vi "Quick Stacks - Image Multi Stacks.vi"(7 "Calling VI Ref":refnum<vi>) -> ()   [LabVIEW 2016]
uses:
  <vilib>/Utility/miscctls.llb/LVPointTypeDef.ctl
  Quick Stacks Type Defs/Quick Stack Marked Areas Actions.ctl
  Quick Stacks Type Defs/Quick Stacks Notifier Type.ctl
  Quick Stacks Type Defs/Quick Stack Actions.ctl
  Hardware Configuration/Hardware Configuration Controls/Device Function.ctl
  Hardware Configuration/Hardware Configuration Controls/Device Type.ctl
  Device Library/Stages/Stages Controls/Stage Actions.ctl
  Quick Stacks Type Defs/Quick Stacks Multi Stack Meta Data.ctl
panel:
  out "Current Delay Time (s)":dbl=1.0 format="%.1f"
  out "Current Cycle":u16=1 min=1
  out "XY Positions":cluster{dbl[], dbl[]}[](graph)
  in  "Cycle Delay (s)":u32
  in  "Number of Cycles":u16=1 min=1
  in  "Capture":bool
  in  "Clear All":bool
  in  "Clear Selected":bool
  in  "Mark Point":bool
  in  "Marked Positions":i32(listbox)
  in  "Quit":bool
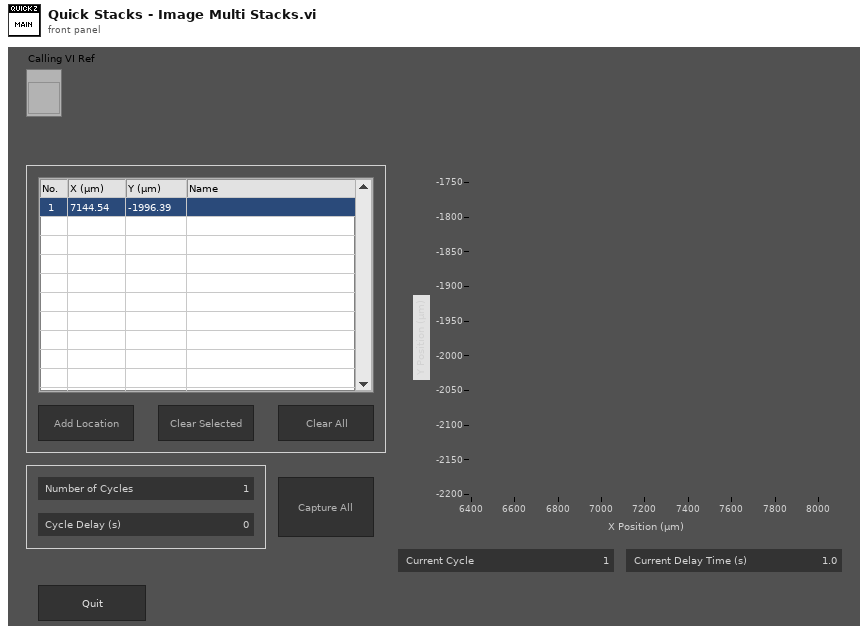
[diagram p1: front panel]
types:
  T1 = typedef "Quick Stacks Notifier Type.ctl" = cluster{"Actions":T2, "Start Z (µm)":dbl, "End Z (µm)":dbl, "Z Size (µm)":dbl, "Num of Steps":u16, "Frames per Step":u16, "Cycle Delay (s)":u32, "Num of Cycles":u16, "Save Path":path, "Running?":bool, "Save File Refs":refnum<file>[]}
  T2 = typedef "Quick Stack Actions.ctl" = enum16{"Idle", "Update Range", "Start Acquisition", "Open File", "Close File", "Start Camera", "Stop Camera", "Laser On", "Laser Off", "Get Image", "Step Z", "Move to Z Start", "Check Cycle", "Abort", "Exit Loop", "Quit"}
  T3 = typedef "Quick Stack Marked Areas Actions.ctl" = enum16{"Add Position", "Update File Name", "Remove Position", "Start Capture", "Move to Position", "Write Meta Data", "Capture", "Switch", "Delay", "Reset Path", "Clear All", "Abort", "Exit Loop", "Quit"}
  T4 = enum16{"Always On", "Always Off", "Off While Running"}
  T5 = typedef "LVPointTypeDef.ctl" = cluster{"Horizontal":i16, "Vertical":i16}
  T6 = typedef "Device Function.ctl" = enum16{"Primary", "Secondary", "Overview", "Wide Field Drift Correction", "642 nm Excitation", "560 nm Excitation", "940 nm Excitation", "546 nm Excitation", "488 nm Excitation", "405 nm Excitation", "Objective Drift Correction", "4Pi Objective Lock", "Objective XY", "Objective Z", "Sample XY", "Sample Coarse Z", "Sample Z", "4Pi Lower", "4Pi Upper", "Mojo", "Adj Cavity", "Line Scanning", "Alert"}
  T7 = typedef "Device Type.ctl" = enum16{"AOTF", "Camera", "Deformable Mirror", "Laser", "Shutter", "Stage", "Waveform", "FPGA", "Email", "Filter Wheel"}
  T8 = typedef "Stage Actions.ctl" = enum16{"Get Position", "MVR", "MOVE", "HALT", "ONTARGET", "ERROR", "REFERENCE", "INIT", "VELOCITY", "STATUS", "EXIT", "HOME", "ZEROPOS", "NANOPOS", "ANALOG", "QUIT"}
  T9 = typedef "Quick Stacks Multi Stack Meta Data.ctl" = cluster{"Start Z (µm)":dbl, "End Z (µm)":dbl, "Z Size (µm)":dbl, "Num of Steps":u16, "Frames per Step":u16, "Cycle Delay (s)":u32, "Num of Cycles":u16}
  T10 = enum32{"Invalid", "Standard", "Closed", "Hidden", "Minimized", "Maximized"}
  T11 = enum8{"Enabled", "Disabled", "Disabled and Grayed Out"}
  T12 = typedef "LVRectTypeDef.ctl" = cluster{"Left":i16, "Top":i16, "Right":i16, "Bottom":i16}
  T13 = typedef "LVBoundsTypeDef.ctl" = cluster{"Width":u32, "Height":u32}
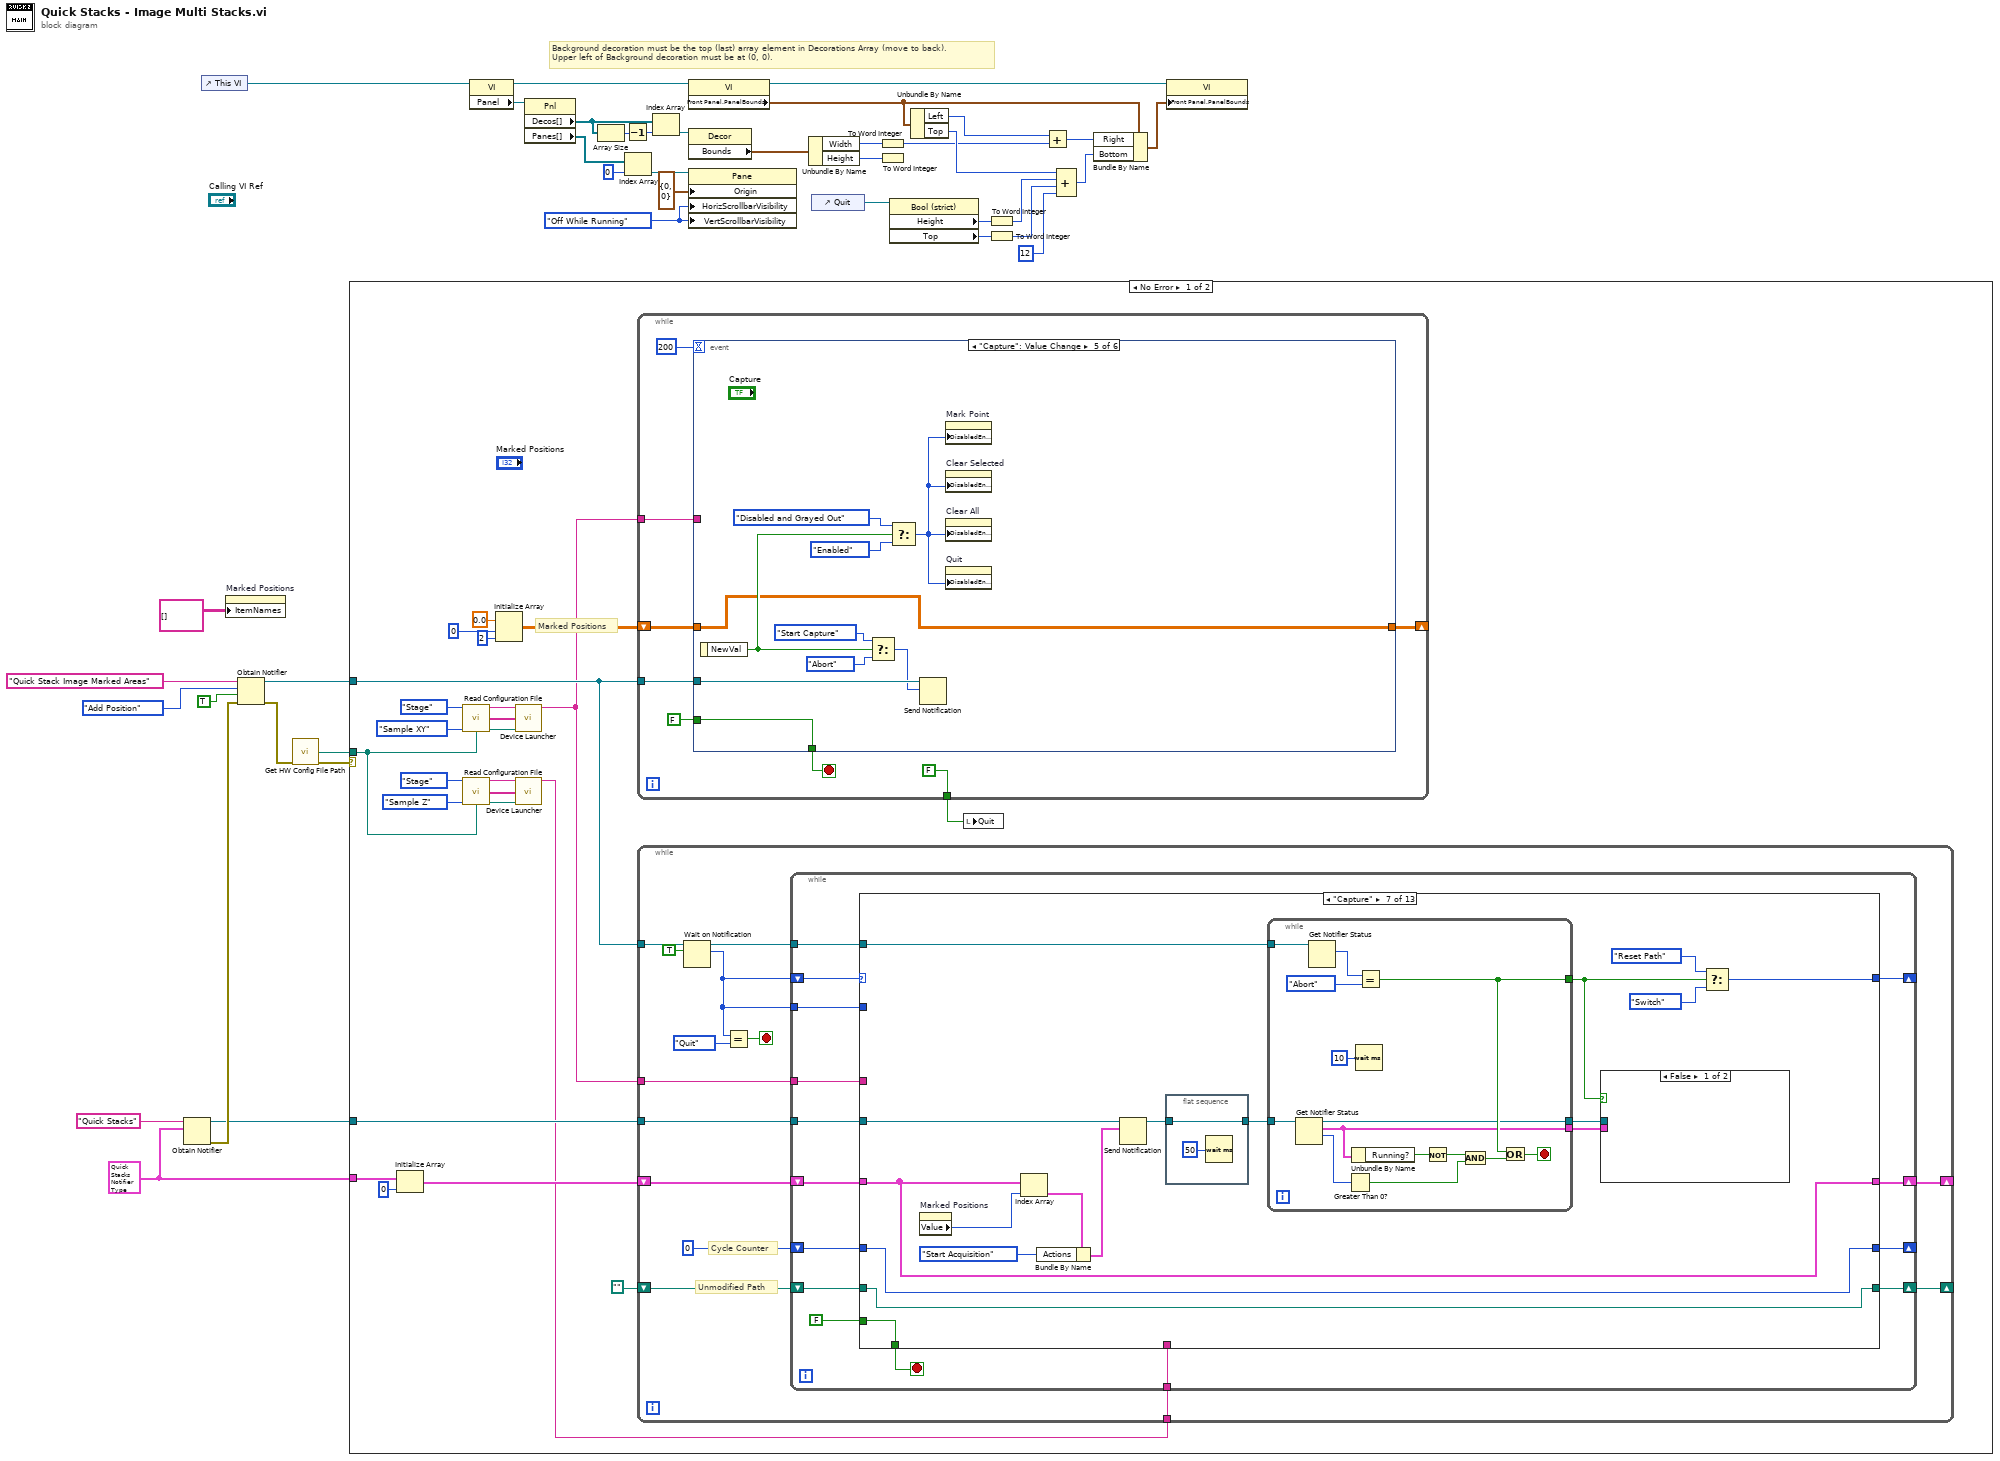
[diagram p0: block diagram]
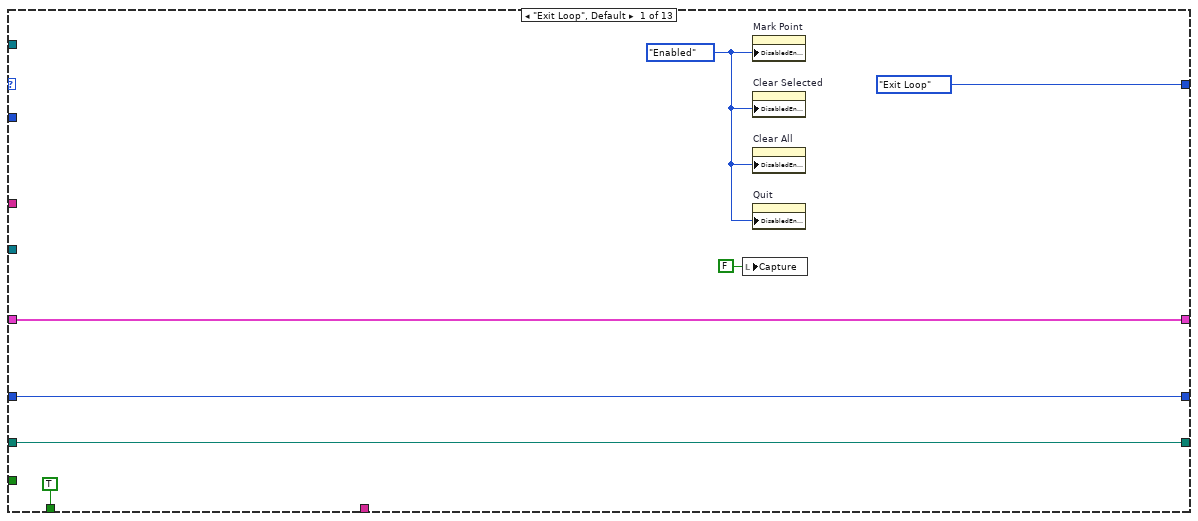
[diagram p2: hidden frame]
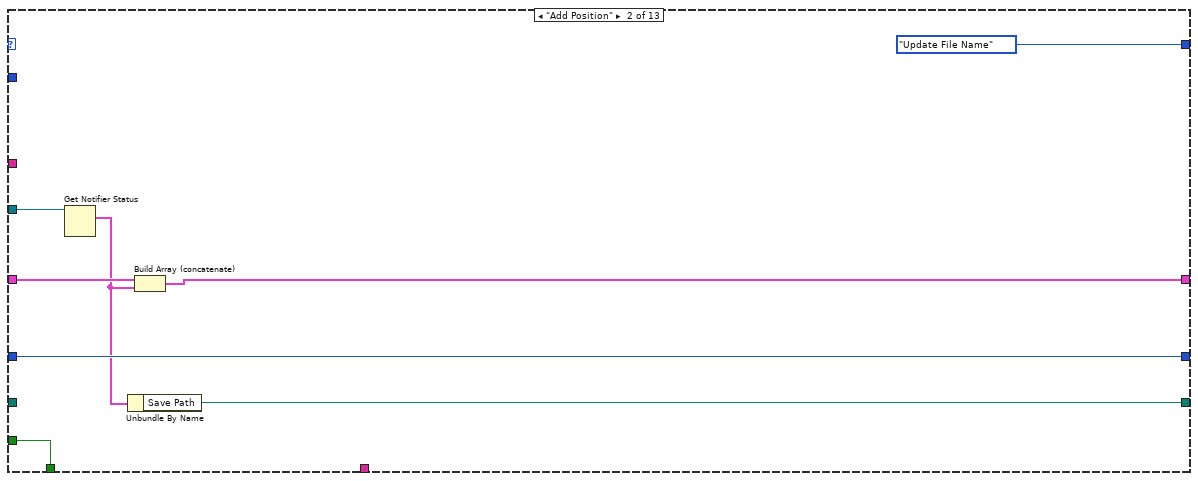
[diagram p3: hidden frame]
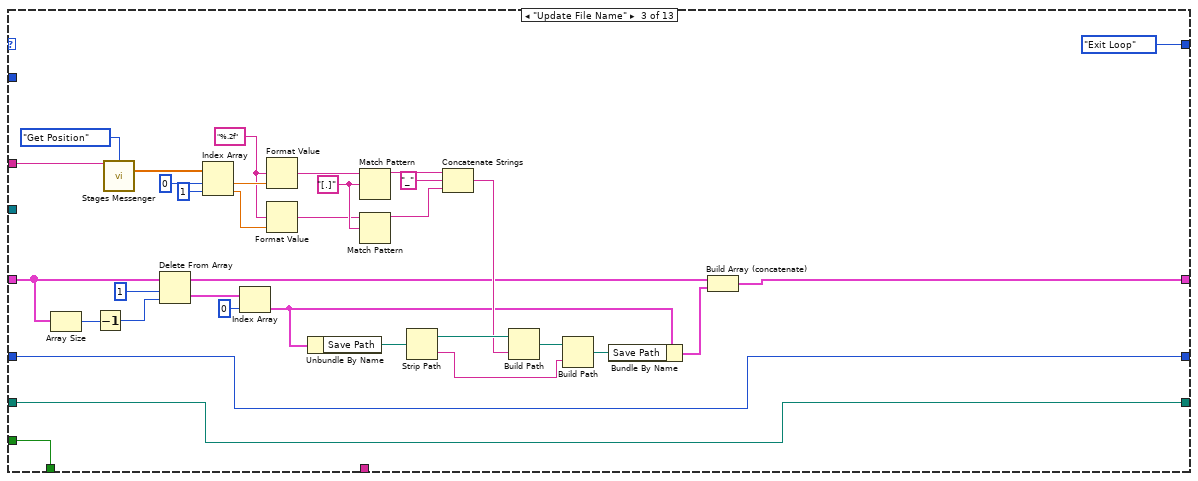
[diagram p4: hidden frame]
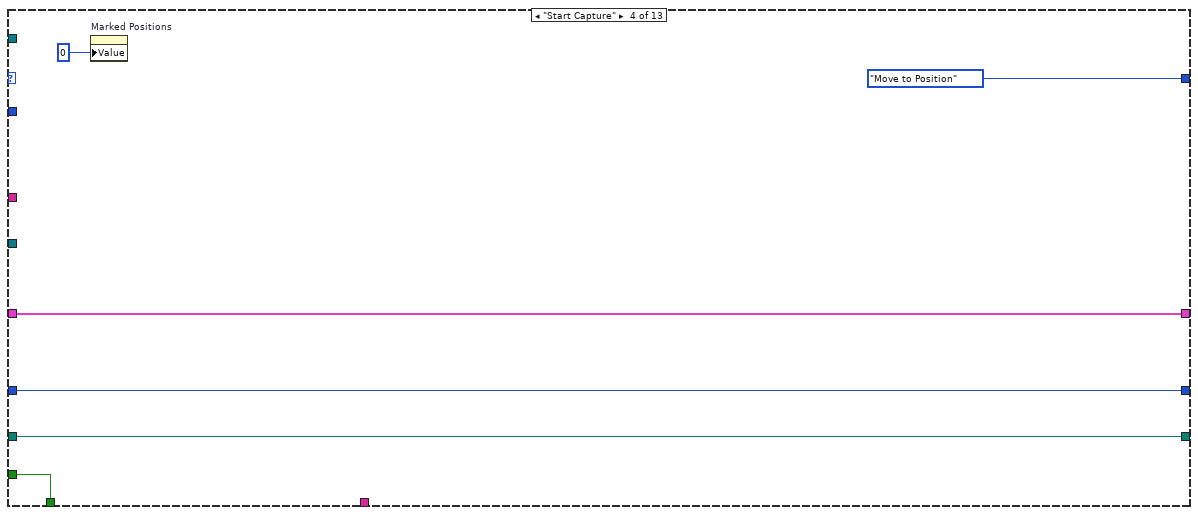
[diagram p5: hidden frame]
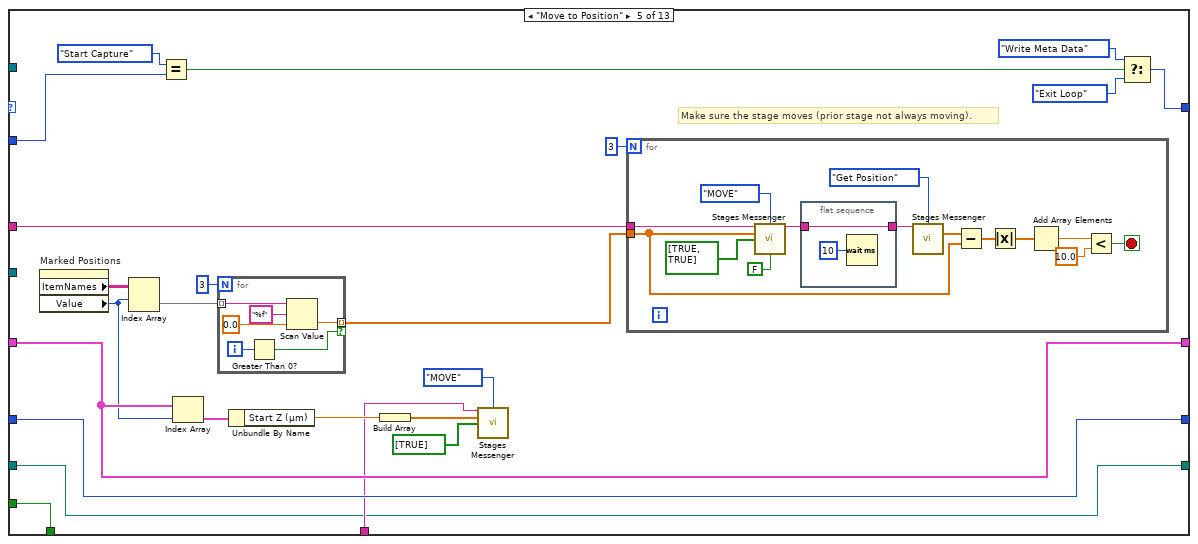
[diagram p6: hidden frame]
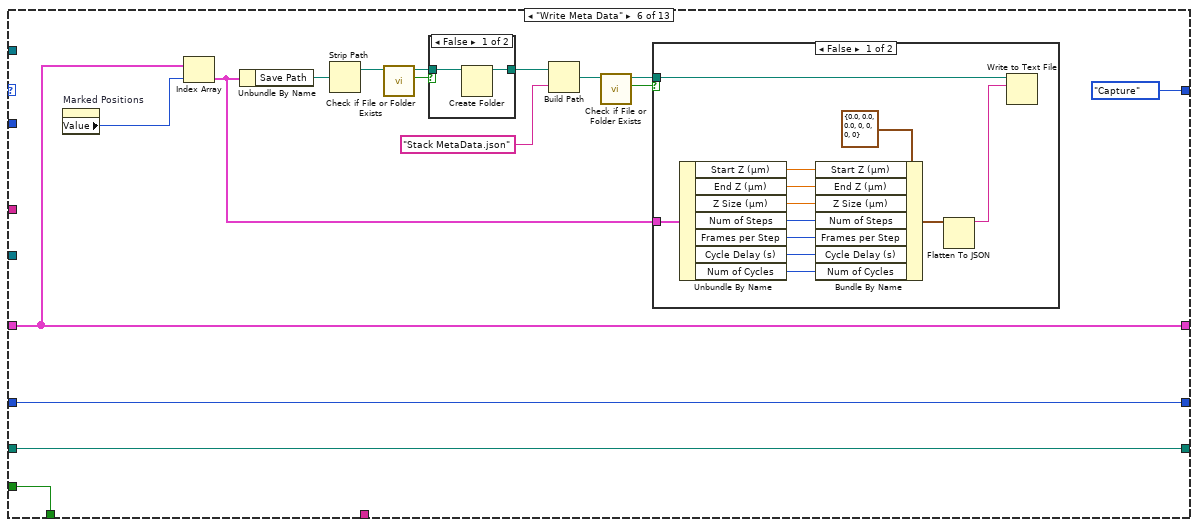
[diagram p7: hidden frame]
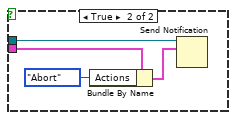
[diagram p10: hidden frame]
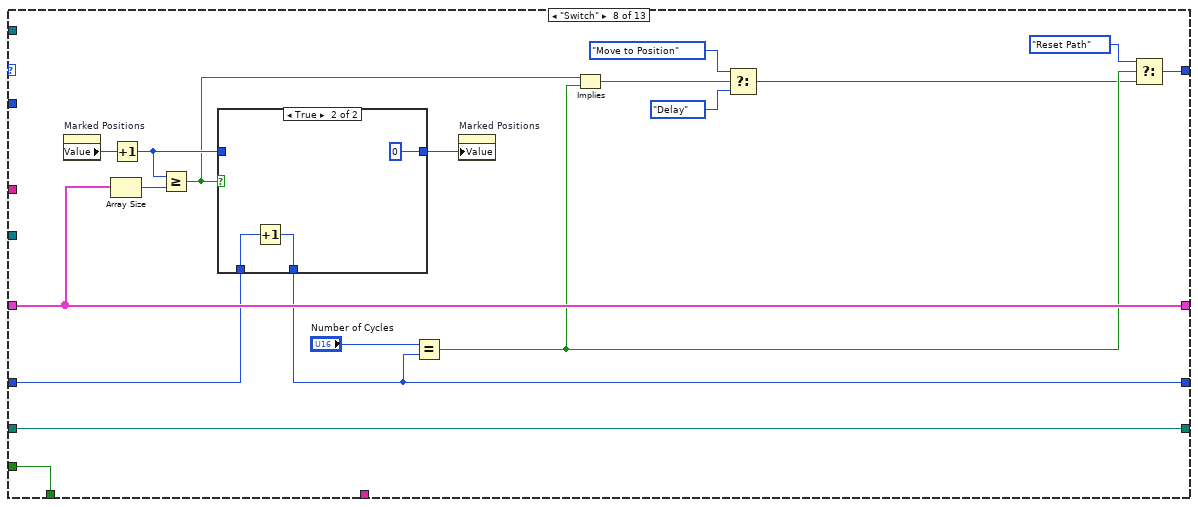
[diagram p11: hidden frame]
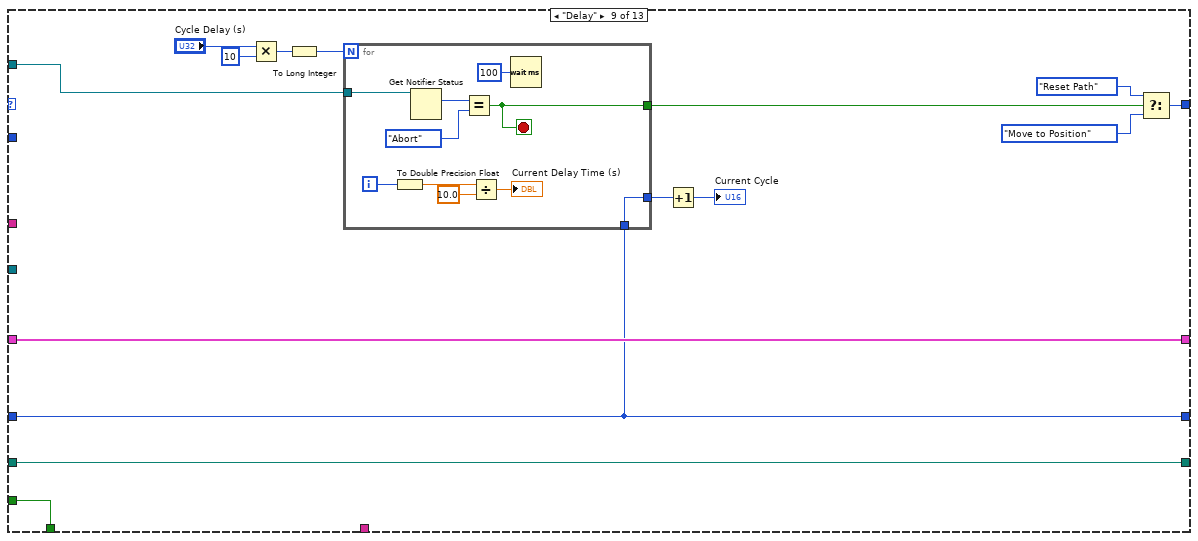
[diagram p13: hidden frame]
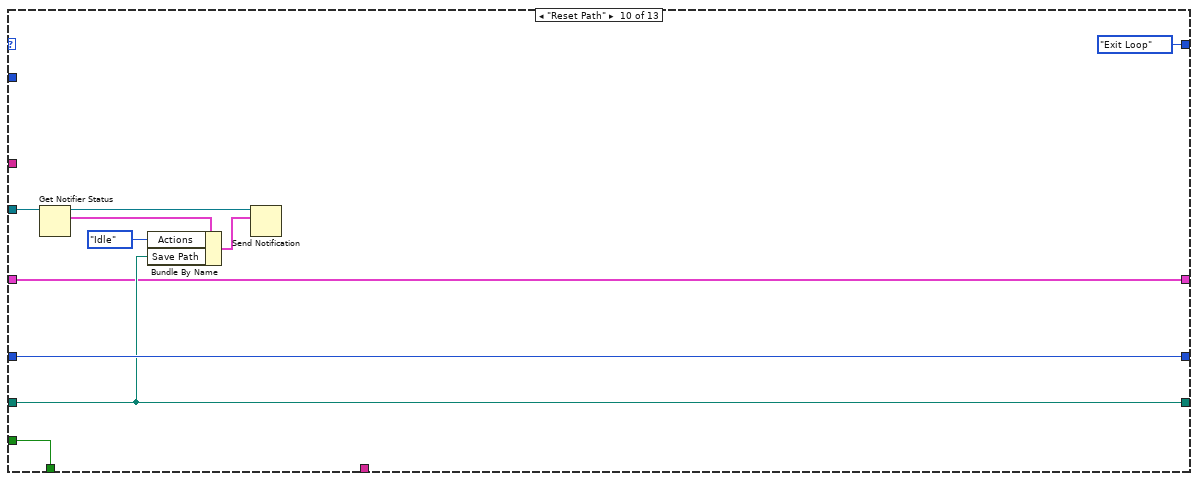
[diagram p14: hidden frame]
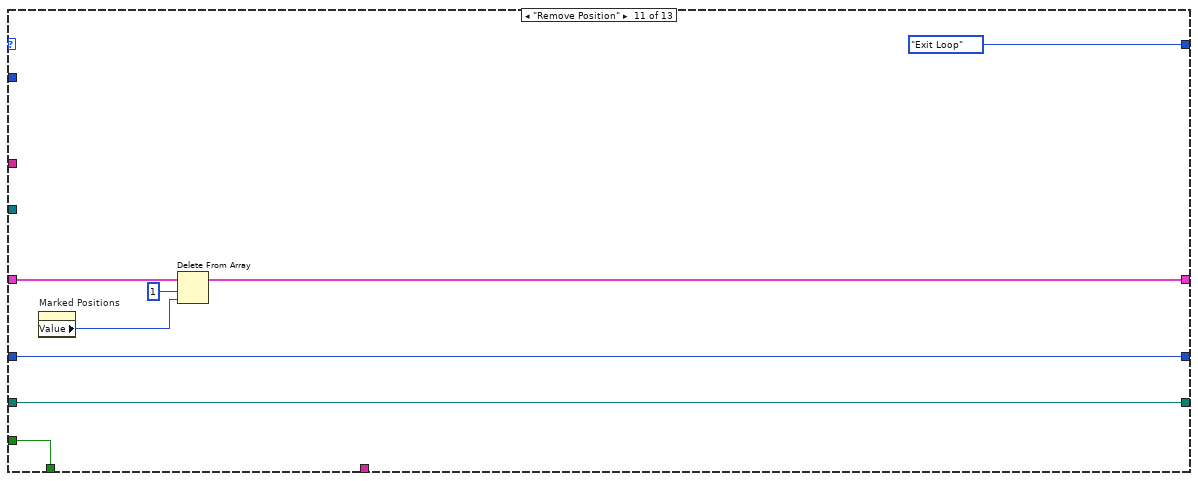
[diagram p15: hidden frame]
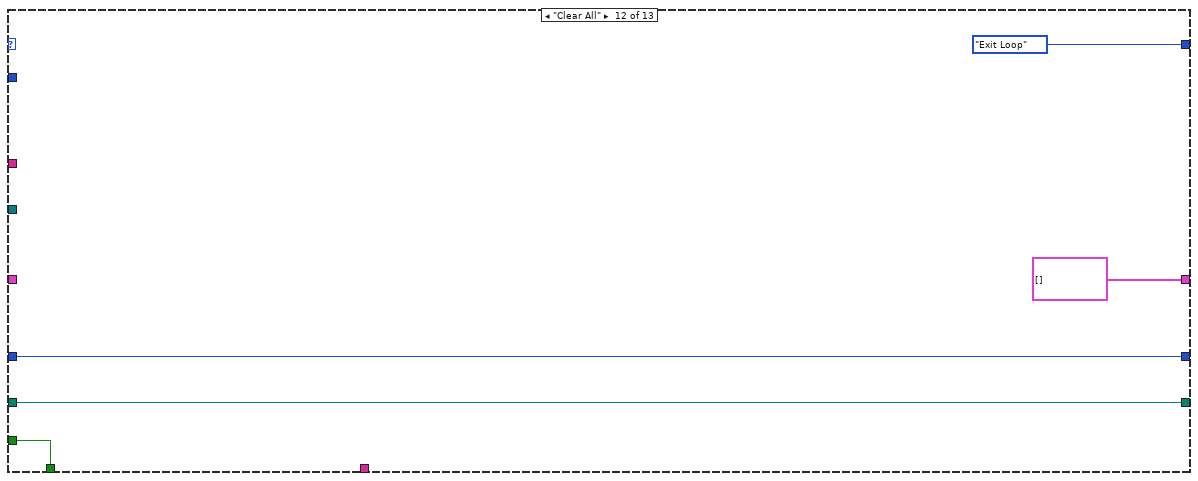
[diagram p16: hidden frame]
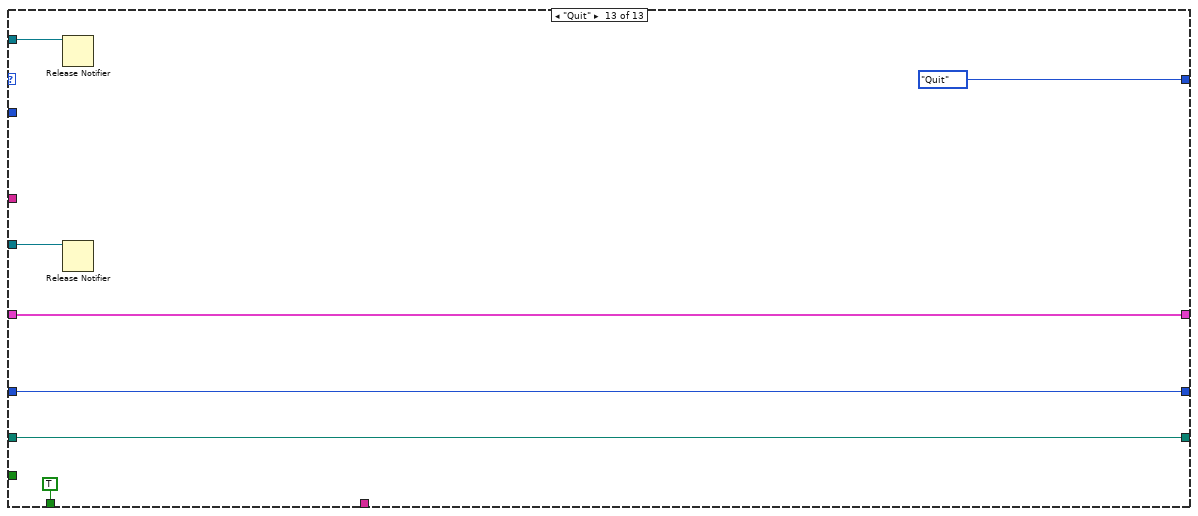
[diagram p17: hidden frame]
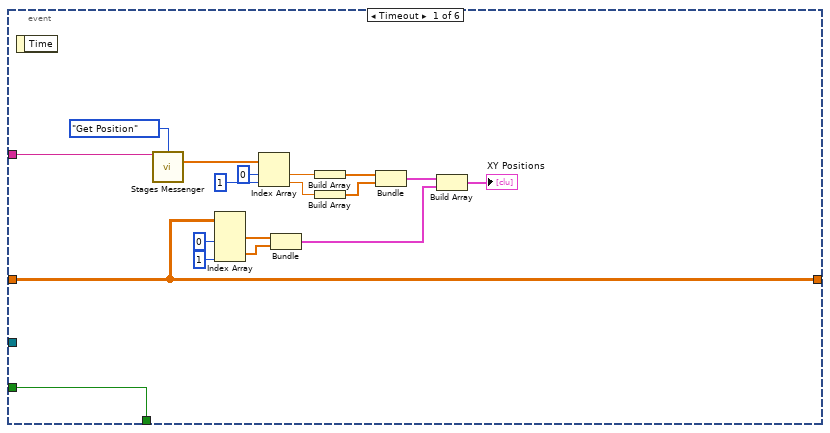
[diagram p18: hidden frame]
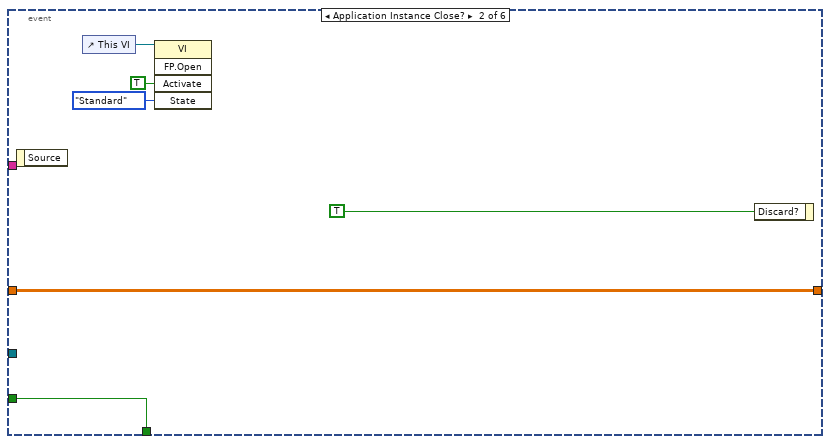
[diagram p19: hidden frame]
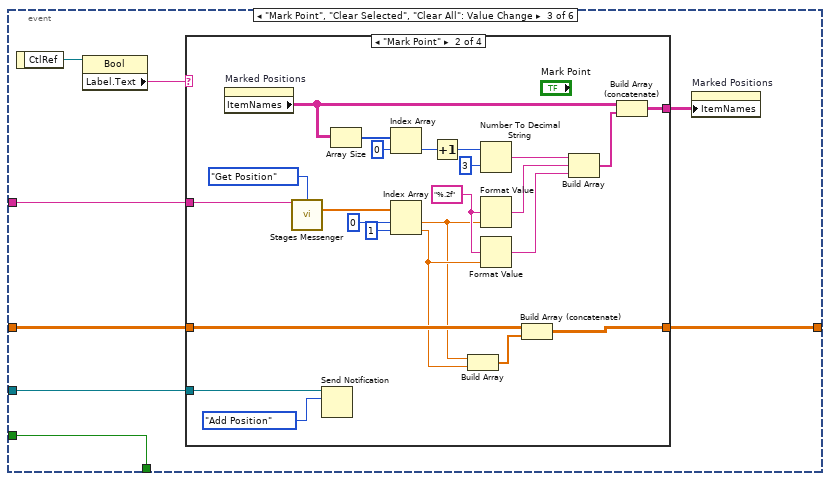
[diagram p20: hidden frame]
diagram:
  w1 = T1 {"Actions"=enum."Idle", "Start Z (µm)"=0.0, "End Z (µm)"=0.0, "Z Size (µm)"=0.0, "Num of Steps"=0, "Frames per Step"=0, "Cycle Delay (s)"=0, "Num of Cycles"=0, "Save Path"=path "", "Running?"=FALSE, "Save File Refs"=[]} ("Stack Parameters")
  w22 = T4."Off While Running" ("Vertical Scrollbar Visibility")
  # "Background decoration must be the top (last) array element in Decorations Array (move to back).\nUpper left of Background decoration must be at (0, 0)."
  n1 = Obtain Notifier(name (unnamed)="Quick Stacks", notification data type=w1) -> (notifier out=w2:refnum<notifier>, error out=w3:errorcluster)  [unwired: 2 in, 1 out]
  n2 = control-ref of="This VI"() -> (w14:refnum<vi>)
  n3 = property on="Marked Positions" class="MCListbox (strict)"("ItemNames"=string[][] [] ("Item Names")) -> ()  [unwired: 2 in, 2 out]
  n4 = Obtain Notifier(name (unnamed)="Quick Stack Image Marked Areas", notification data type=Quick_Stack_Marked_Areas_Actions."Add Position" ("Actions"), create if not found? (T)=TRUE, error in (no error)=w3) -> (notifier out=w7:refnum<notifier>, error out=w8:errorcluster)  [unwired: 1 out]
  n5 = call "Get HW Config File Path.vi"("Error"=w8) -> ("File Path"=w40:path, "Error"=w41:errorcluster)  [unwired: 13 in]
  n6 = case shown="No Error" w41 {
    tunnel: w40 -> [w44 _]
    tunnel: w7 -> [w59 _]
    tunnel: w2 -> [w57 _]
    tunnel: w1 -> [w56 _]
    frame No Error {
      # "Marked Positions"
      n7 = Initialize Array(w56, 0 ("dimension size")) -> (w54:T1[])
      n8 = call "Read Configuration File.vi"("Device Type"=Device_Type."Stage", "Device Function"=Device_Function."Sample XY", "Config File Path"=w44) -> ("Unique Notifier Name"=w63:string, "Device Ports/IDs/Channels"=w65:string[], "Device Engine Path"=w64:path)  [unwired: 9 in, 1 out]
      n9 = call "Read Configuration File.vi"("Device Type"=Device_Type."Stage", "Device Function"=Device_Function."Sample Z", "Config File Path"=w44) -> ("Unique Notifier Name"=w47:string, "Device Ports/IDs/Channels"=w45:string[], "Device Engine Path"=w46:path)  [unwired: 9 in, 1 out]
      n10 = Initialize Array(0.0 ("element"), 0 ("dimension size"), 2 ("dimension size")) -> (w52:dbl[][])
      n11 = call "Device Launcher.vi"("Notifier Name"=w63, "Device Ports/IDs/Channels"=w65, "Device Engine Path"=w64) -> ("Notifier Name"=w58:string)  [unwired: 11 in, 1 out]
      n12 = call "Device Launcher.vi"("Notifier Name"=w47, "Device Ports/IDs/Channels"=w45, "Device Engine Path"=w46) -> ("Notifier Name"=w43:string)  [unwired: 11 in, 1 out]
      n13 = while {
        tunnel: [FALSE] -> w60
        tunnel: w58 -> [w345]
        tunnel: w59 -> [w344]
        shift-right: [w342] -> _
        shift-left: w52 -> [w343]
        stop <- w347 stop-if-true
        n14 = event shown="[4] \"Capture\": Value Change" {
          selector: _ -> [_ _ _ _ _ _]
          dyn-events: _ -> [_ _ _ _ _ _]
          timeout: 200 -> [_ _ _ _ _ _]
          tunnel: FALSE -> [w367 w372 w381 w433 w443 _]
          tunnel: [w367 w372 w381 w433 w443 w447] -> w347
          tunnel: w345 -> [w365 _ w378 _ _ _]
          tunnel: w344 -> [_ _ w376 w432 w442 w446]
          tunnel: w343 -> [w357 w368 w375 w430 w434 w444]
          tunnel: [w357 w368 w374 w430 w434 w444] -> w342
          event Timeout {
            n15 = event-data() -> ()  [unwired: 1 in, 1 out]
            n16 = call "Stages Messenger.vi"("Stage Notifier Name"=w365, "Actions"=Stage_Actions."Get Position") -> ("Positions"=w364:dbl[])  [unwired: 10 in, 3 out]
            n17 = Index Array(array=w357, index (col) #1=0 ("disabled index (col)"), index (col) #2=1 ("index (col)")) -> (element #1=w354:dbl[], element #2=w353:dbl[])  [unwired: 2 in]
            n18 = Index Array(array=w364, index #1=0 ("index"), index #2=1 ("index")) -> (element #1=w361:dbl, element #2=w360:dbl)
            n19 = Bundle(w354, w353) -> (w351:cluster{dbl[], dbl[]})  [unwired: 1 in]
            n20 = Build Array(w361) -> (w359:dbl[])
            n21 = Build Array(w360) -> (w358:dbl[])
            n22 = Bundle(w359, w358) -> (w352:cluster{dbl[], dbl[]})  [unwired: 1 in]
            n23 = Build Array(w352, w351) -> (→"XY Positions":cluster{dbl[], dbl[]}[])
          }
          event Application Instance Close? {
            n24 = event-data() -> ()  [unwired: 1 in, 1 out]
            n25 = control-ref of="This VI"() -> (w369:refnum<vi>)
            n26 = invoke class="VI" method="FP.Open"(reference=w369, "Activate"=TRUE ("Activate?"), "State"=T10."Standard") -> ()  [unwired: 2 in, 5 out]
            n27 = event-data("Discard?"=TRUE) -> ()  [unwired: 1 in, 1 out]
          }
          event "Mark Point", "Clear Selected", "Clear All": Value Change {
            n28 = event-data() -> ("CtlRef"=w380:refnum<vi>)  [unwired: 1 in]
            n29 = property class="Bool"(reference=w380) -> ("Label.Text"=w377:string)  [unwired: 1 in, 2 out]
            n30 = case shown="\"Mark Point\"" w377 {
              tunnel: [w385 w396 w419 string[][] []] -> w379
              tunnel: w378 -> [_ w394 _ _]
              tunnel: w376 -> [w384 w392 w417 w428]
              tunnel: w375 -> [w382 w390 w413 _]
              tunnel: [w382 w386 w411 w423] -> w374
              frame Default {
                n31 = Send Notification(notification=Quick_Stack_Marked_Areas_Actions."Exit Loop", notifier=w384) -> ()  [unwired: 1 in, 2 out]
                n32 = property on="Marked Positions" class="MCListbox (strict)"() -> ("ItemNames"=w385:string[][])  [unwired: 2 in, 2 out]
              }
              frame "Mark Point" {
                w393 = "%.2f" ("format string")
                n33 = property on="Marked Positions" class="MCListbox (strict)"() -> ("ItemNames"=w398:string[][])  [unwired: 2 in, 2 out]
                n34 = call "Stages Messenger.vi"("Stage Notifier Name"=w394, "Actions"=Stage_Actions."Get Position") -> ("Positions"=w395:dbl[])  [unwired: 10 in, 3 out]
                n35 = Send Notification(notification=Quick_Stack_Marked_Areas_Actions."Add Position", notifier=w392) -> ()  [unwired: 1 in, 2 out]
                n36 = Array Size(array=w398) -> (size(s)=w404:i32[])
                n37 = Index Array(array=w404, index=0) -> (element=w402:i32)
                n38 = Index Array(array=w395, index #1=0 ("index"), index #2=1 ("index")) -> (element #1=w388:dbl, element #2=w389:dbl)
                n39 = Increment(x=w402) -> (x+1=w406:i32)
                n40 = Build Array(w388, w389) -> (w387:dbl[])
                n41 = Number To Decimal String(number=w406, width (-)=i16 3) -> (decimal integer string=w401:string)
                n42 = Format Value(format string=w393, value (0)=w388) -> (output string=w399:string)  [unwired: 1 in]
                n43 = Format Value(format string=w393, value (0)=w389) -> (output string=w400:string)  [unwired: 1 in]
                n44 = Build Array (concatenate)(w390, w387) -> (w386:dbl[][])
                n45 = Build Array(w401, w399, w400) -> (w397:string[])
                n46 = Build Array (concatenate)(w398, w397) -> (w396:string[][])
              }
              frame "Clear Selected" {
                n47 = Send Notification(notification=Quick_Stack_Marked_Areas_Actions."Remove Position", notifier=w417) -> (error out=w415:errorcluster)  [unwired: 1 in, 1 out]
                n48 = flat-sequence {
                  tunnel: w415 -> [w421]
                  tunnel: [w421] -> w414
                  frame #0 {
                    n49 = Wait (ms)(milliseconds to wait=u32 10) -> ()  [unwired: 1 out]
                  }
                }
                n50 = property on="Marked Positions" class="MCListbox (strict)"() -> ("ItemNames"=w420:string[][])  [unwired: 2 in, 2 out]
                n51 = property on="Marked Positions" class="MCListbox (strict)"(error in=w414) -> ("Value"=w412:i32)  [unwired: 1 in, 2 out]
                n52 = Delete From Array(array=w420, length=1, index (row)=w412) -> (array with subset deleted=w419:string[][])  [unwired: 1 in, 1 out]
                n53 = Delete From Array(array=w413, length=1, index (row)=w412) -> (array with subset deleted=w411:dbl[][])  [unwired: 1 in, 1 out]
              }
              frame "Clear All" {
                n54 = Send Notification(notification=Quick_Stack_Marked_Areas_Actions."Clear All", notifier=w428) -> ()  [unwired: 1 in, 2 out]
                n55 = Initialize Array(0.0 ("element"), 0 ("dimension size"), 2 ("dimension size")) -> (w423:dbl[][])
              }
            }
            n56 = property on="Marked Positions" class="MCListbox (strict)"("ItemNames"=w379) -> ()  [unwired: 2 in, 2 out]
          }
          event "Marked Positions": Double Click {
            n57 = event-data() -> ()  [unwired: 1 in, 1 out]
            n58 = Send Notification(notification=Quick_Stack_Marked_Areas_Actions."Move to Position", notifier=w432) -> ()  [unwired: 1 in, 2 out]
          }
          event "Capture": Value Change {
            n59 = event-data() -> ("NewVal"=w439:bool)  [unwired: 1 in]
            n60 = Select(t=Quick_Stack_Marked_Areas_Actions."Start Capture", s=w439, f=Quick_Stack_Marked_Areas_Actions."Abort" ("y")) -> (s? t:f=w440:T3)
            n61 = Select(t=T11."Disabled and Grayed Out" ("Disabled"), s=w439, f=T11."Enabled" ("Disabled")) -> (s? t:f=w436:T11)
            n62 = Send Notification(notification=w440, notifier=w442) -> ()  [unwired: 1 in, 2 out]
            n63 = property on="Mark Point" class="Bool"("DisabledEnum"=w436) -> ()  [unwired: 2 in, 2 out]
            n64 = property on="Clear Selected" class="Bool"("DisabledEnum"=w436) -> ()  [unwired: 2 in, 2 out]
            n65 = property on="Clear All" class="Bool"("DisabledEnum"=w436) -> ()  [unwired: 2 in, 2 out]
            n66 = property on="Quit" class="Bool (strict)"("DisabledEnum"=w436) -> ()  [unwired: 2 in, 2 out]
          }
          event "Quit": Value Change {
            n67 = event-data() -> ("NewVal"=w447:bool)  [unwired: 1 in]
            n68 = Send Notification(notification=Quick_Stack_Marked_Areas_Actions."Quit", notifier=w446) -> ()  [unwired: 1 in, 2 out]
          }
        }
      }
      n69 = while {
        tunnel: w59 -> [w79]
        tunnel: w58 -> [w73]
        tunnel: w57 -> [w72]
        shift-right: [w70] -> _
        shift-left: w54 -> [w71]
        tunnel: w43 -> [w68]
        shift-right: [w67] -> _
        shift-left: path "" -> [w66]
        stop <- w76 stop-if-true
        # "Unmodified Path"
        # "Cycle Counter"
        n70 = Wait on Notification(notifier=w79, ignore previous (F)=TRUE) -> (notifier out=w75:refnum<notifier>, notification=w74:T3)  [unwired: 2 in, 2 out]
        n71 = Equal?(x=w74, y=Quick_Stack_Marked_Areas_Actions."Quit") -> (x = y?=w76:bool)
        n72 = while {
          shift-right: [w90] -> _
          shift-left: w74 -> [w93]
          tunnel: w75 -> [w94]
          tunnel: w74 -> [w89]
          tunnel: w73 -> [w88]
          tunnel: w72 -> [w87]
          shift-right: [w85] -> w70
          shift-left: w71 -> [w86]
          shift-right: [w83] -> _
          shift-left: u16 0 -> [w84]
          tunnel: w68 -> [w82]
          shift-right: [w81] -> w67
          shift-left: w66 -> [w80]
          stop <- w91 stop-if-true
          n73 = case shown="\"Capture\"" w93 {
            tunnel: w94 -> [_ _ _ _ _ _ w242 _ w292 _ _ _ w339]
            tunnel: [TRUE w109 w143 w149 w172 w209 w243 w281 w301 w320 w328 w333 TRUE] -> w91
            tunnel: FALSE -> [_ w109 w143 w149 w172 w209 w243 w281 w301 w320 w328 w333 _]
            tunnel: [Quick_Stack_Marked_Areas_Actions."Exit Loop" ("y") Quick_Stack_Marked_Areas_Actions."Update File Name" ("y") Quick_Stack_Marked_Areas_Actions."Exit Loop" ("y") Quick_Stack_Marked_Areas_Actions."Move to Position" ("y") w166 Quick_Stack_Marked_Areas_Actions."Capture" ("y") w240 w277 w293 Quick_Stack_Marked_Areas_Actions."Exit Loop" ("y") Quick_Stack_Marked_Areas_Actions."Exit Loop" ("y") Quick_Stack_Marked_Areas_Actions."Exit Loop" ("y") Quick_Stack_Marked_Areas_Actions."Quit" ("y")] -> w90
            tunnel: w89 -> [_ _ _ _ w169 _ _ _ _ _ _ _ _]
            tunnel: w88 -> [_ _ w123 _ w163 _ _ _ _ _ _ _ _]
            tunnel: w87 -> [_ w107 _ _ _ _ w235 _ _ w318 _ _ w338]
            tunnel: w86 -> [w97 w106 w132 w146 w159 w197 w232 w276 w300 w312 w325 _ w337]
            tunnel: [w97 w105 w114 w146 w159 w197 w232 w276 w300 w312 w324 T1[] [] w337] -> w85
            tunnel: w84 -> [w96 w104 w139 w145 w160 w208 w228 w273 w290 w321 w323 w331 w336]
            tunnel: [w96 w104 w139 w145 w160 w208 w228 w271 w290 w321 w323 w331 w336] -> w83
            tunnel: w82 -> [_ _ _ _ w152 _ _ _ _ _ _ _ _]
            tunnel: [w95 w102 w110 w144 w151 w195 w226 w264 w287 w313 w322 w330 w335] -> w81
            tunnel: w80 -> [w95 _ w110 w144 w151 w195 w226 w264 w287 w313 w322 w330 w335]
            frame "Exit Loop", Default {
              w99 = T11."Enabled" ("Disabled")
              n74 = local write "Capture"(FALSE ("Capture")) -> ()
              n75 = property on="Mark Point" class="Bool"("DisabledEnum"=w99) -> ()  [unwired: 2 in, 2 out]
              n76 = property on="Clear Selected" class="Bool"("DisabledEnum"=w99) -> ()  [unwired: 2 in, 2 out]
              n77 = property on="Clear All" class="Bool"("DisabledEnum"=w99) -> ()  [unwired: 2 in, 2 out]
              n78 = property on="Quit" class="Bool (strict)"("DisabledEnum"=w99) -> ()  [unwired: 2 in, 2 out]
            }
            frame "Add Position" {
              n79 = Get Notifier Status(notifier=w107) -> (current notification=w103:T1)  [unwired: 1 in, 4 out]
              n80 = Unbundle By Name(w103) -> ("Save Path"=w102:path)
              n81 = Build Array (concatenate)(w106, w103) -> (w105:T1[])
            }
            frame "Update File Name" {
              w124 = "%.2f" ("format string")
              w138 = "[.]" ("regular expression")
              n82 = Array Size(array=w132) -> (size(s)=w133:i32)
              n83 = Decrement(x=w133) -> (x-1=w130:i32)
              n84 = call "Stages Messenger.vi"("Stage Notifier Name"=w123, "Actions"=Stage_Actions."Get Position") -> ("Positions"=w125:dbl[])  [unwired: 10 in, 3 out]
              n85 = Delete From Array(array=w132, length=1, index=w130) -> (deleted portion=w118:T1[], array with subset deleted=w119:T1[])
              n86 = Index Array(array=w125, index #1=0 ("index"), index #2=1 ("index")) -> (element #1=w127:dbl, element #2=w126:dbl)
              n87 = Index Array(array=w118, index=0) -> (element=w116:T1)
              n88 = Format Value(format string=w124, value (0)=w127) -> (output string=w121:string)  [unwired: 1 in]
              n89 = Format Value(format string=w124, value (0)=w126) -> (output string=w120:string)  [unwired: 1 in]
              n90 = Unbundle By Name(w116) -> ("Save Path"=w142:path)
              n91 = Match Pattern(string=w121, regular expression=w138) -> (before substring=w137:string)  [unwired: 1 in, 3 out]
              n92 = Match Pattern(string=w120, regular expression=w138) -> (before substring=w136:string)  [unwired: 1 in, 3 out]
              n93 = Strip Path(path=w142) -> (stripped path=w141:path, name=w112:string)
              n94 = Concatenate Strings(w137, "_" ("string"), w136) -> (w134:string)
              n95 = Build Path(base path=w141, name or relative path=w134) -> (appended path=w113:path)
              n96 = Build Path(base path=w113, name or relative path=w112) -> (appended path=w111:path)
              n97 = Bundle By Name(cluster=w116, "Save Path"=w111) -> (w115:T1)
              n98 = Build Array (concatenate)(w119, w115) -> (w114:T1[])
            }
            frame "Start Capture" {
              n99 = property on="Marked Positions" class="MCListbox (strict)"("Value"=0 ("Focus Row")) -> ()  [unwired: 2 in, 2 out]
            }
            frame "Move to Position" {
              # "Make sure the stage moves (prior stage not always moving)."
              n100 = property on="Marked Positions" class="MCListbox (strict)"() -> ("ItemNames"=w165:string[][], "Value"=w158:i32)  [unwired: 2 in, 2 out]
              n101 = Index Array(array=w165, index (row)=w158) -> (element=w164:string[])  [unwired: 1 in]
              n102 = Equal?(x=Quick_Stack_Marked_Areas_Actions."Start Capture" ("y"), y=w169) -> (x = y?=w171:bool)
              n103 = Index Array(array=w159, index=w158) -> (element=w157:T1)
              n104 = for {
                N: 3 -> [_]
                tunnel: w164 -> [w192] mode=indexing
                tunnel: [w191] -> w162 mode=indexing if=w189
                i -> [w190]
                n105 = Greater Than 0?(x=w190) -> (x > 0?=w189:bool)
                n106 = Scan Value(string=w192, format string="%f", default (0 dbl)=0.0) -> (value=w191:dbl)  [unwired: 1 out]
              }
              n107 = Unbundle By Name(w157) -> ("Start Z (µm)"=w155:dbl)
              n108 = Build Array(w155) -> (w154:dbl[])
              n109 = call "Stages Messenger.vi"("Stage Notifier Name"=w152, "Actions"=Stage_Actions."MOVE", "Setpoint"=w154, "Axis"=bool[] [TRUE]) -> ()  [unwired: 8 in, 4 out]
              n110 = for {
                N: 3 -> [_]
                tunnel: w163 -> [w183]
                tunnel: w162 -> [w178]
                stop <- w173 stop-if-true
                n111 = call "Stages Messenger.vi"("Stage Notifier Name"=w183, "Actions"=Stage_Actions."MOVE", "Setpoint"=w178, "Axis"=bool[] [TRUE, TRUE], "Exit While Busy?"=FALSE ("Wait for On Target? (F)")) -> ("Stage Notifier Name (Dup)"=w182:string)  [unwired: 7 in, 3 out]
                n112 = flat-sequence {
                  tunnel: w182 -> [w187]
                  tunnel: [w187] -> w180
                  frame #0 {
                    n113 = Wait (ms)(milliseconds to wait=u32 10) -> ()  [unwired: 1 out]
                  }
                }
                n114 = call "Stages Messenger.vi"("Stage Notifier Name"=w180, "Actions"=Stage_Actions."Get Position") -> ("Positions"=w179:dbl[])  [unwired: 10 in, 3 out]
                n115 = Subtract(x=w179, y=w178) -> (x-y=w177:dbl[])
                n116 = Absolute Value(x=w177) -> (abs(x)=w176:dbl[])
                n117 = Add Array Elements(numeric array=w176) -> (sum=w175:dbl)
                n118 = Less?(x=w175, y=10.0) -> (x < y?=w173:bool)
              }
              n119 = Select(t=Quick_Stack_Marked_Areas_Actions."Write Meta Data", s=w171, f=Quick_Stack_Marked_Areas_Actions."Exit Loop" ("y")) -> (s? t:f=w166:T3)
            }
            frame "Write Meta Data" {
              n120 = property on="Marked Positions" class="MCListbox (strict)"() -> ("Value"=w207:i32)  [unwired: 2 in, 2 out]
              n121 = Index Array(array=w197, index=w207) -> (element=w196:T1)
              n122 = Unbundle By Name(w196) -> ("Save Path"=w206:path)
              n123 = Strip Path(path=w206) -> (stripped path=w201:path)  [unwired: 1 out]
              n124 = call <vilib>:"Check if File or Folder Exists.vi"("path"=w201) -> ("file or folder exists?"=w200:bool, "dup path"=w199:path)  [unwired: 8 in, 1 out]
              n125 = case shown="False" w200 {
                tunnel: w199 -> [w212 w213]
                tunnel: [w211 w213] -> w198
                frame False {
                  n126 = Create Folder(path (use dialog)=w212) -> (created path=w211:path)  [unwired: 2 in, 2 out]
                }
                frame True {
                }
              }
              n127 = Build Path(base path=w198, name or relative path="Stack MetaData.json") -> (appended path=w204:path)
              n128 = call <vilib>:"Check if File or Folder Exists.vi"("path"=w204) -> ("file or folder exists?"=w203:bool, "dup path"=w202:path)  [unwired: 8 in, 1 out]
              n129 = case shown="False" w203 {
                tunnel: w202 -> [w225 _]
                tunnel: w196 -> [w216 _]
                frame False {
                  n130 = Unbundle By Name(w216) -> ("Start Z (µm)"=w218:dbl, "End Z (µm)"=w219:dbl, "Z Size (µm)"=w220:dbl, "Num of Steps"=w221:u16, "Frames per Step"=w222:u16, "Cycle Delay (s)"=w223:u32, "Num of Cycles"=w214:u16)
                  n131 = Bundle By Name(cluster=T9 {"Start Z (µm)"=0.0, "End Z (µm)"=0.0, "Z Size (µm)"=0.0, "Num of Steps"=0, "Frames per Step"=0, "Cycle Delay (s)"=0, "Num of Cycles"=0} ("Stack Parameters"), "Start Z (µm)"=w218, "End Z (µm)"=w219, "Z Size (µm)"=w220, "Num of Steps"=w221, "Frames per Step"=w222, "Cycle Delay (s)"=w223, "Num of Cycles"=w214) -> (w224:T9)
                  n132 = Flatten To JSON(anything=w224) -> (JSON string=w215:string)  [unwired: 2 in, 1 out]
                  n133 = Write to Text File(file (use dialog)=w225, text=w215) -> ()  [unwired: 2 in, 3 out]
                }
                frame True {
                }
              }
            }
            frame "Capture" {
              n134 = property on="Marked Positions" class="MCListbox (strict)"() -> ("Value"=w238:i32)  [unwired: 2 in, 2 out]
              n135 = Index Array(array=w232, index=w238) -> (element=w239:T1)
              n136 = Bundle By Name(cluster=w239, "Actions"=Quick_Stack_Actions."Start Acquisition") -> (w236:T1)
              n137 = Send Notification(notification=w236, notifier=w235) -> (notifier out=w234:refnum<notifier>)  [unwired: 1 in, 1 out]
              n138 = flat-sequence {
                tunnel: w234 -> [w249]
                tunnel: [w249] -> w233
                frame #0 {
                  n139 = Wait (ms)(milliseconds to wait=u32 50) -> ()  [unwired: 1 out]
                }
              }
              n140 = while {
                tunnel: w242 -> [w263]
                tunnel: [w261] -> w231
                tunnel: w233 -> [w258]
                tunnel: [w252] -> w230
                tunnel: [w251] -> w229
                stop <- w262 stop-if-true
                n141 = Get Notifier Status(notifier=w258) -> (notifier out=w252:refnum<notifier>, current notification=w251:T1, # waiting=w257:i32)  [unwired: 1 in, 2 out]
                n142 = Get Notifier Status(notifier=w263) -> (current notification=w250:T3)  [unwired: 1 in, 4 out]
                n143 = Greater Than 0?(x=w257) -> (x > 0?=w254:bool)
                n144 = Unbundle By Name(w251) -> ("Running?"=w256:bool)
                n145 = Wait (ms)(milliseconds to wait=u32 10) -> ()  [unwired: 1 out]
                n146 = Equal?(x=w250, y=Quick_Stack_Marked_Areas_Actions."Abort") -> (x = y?=w261:bool)
                n147 = Not(x=w256) -> (.not. x?=w255:bool)
                n148 = And(x=w255, y=w254) -> (x .and. y?=w253:bool)
                n149 = Or(x=w261, y=w253) -> (x .or. y?=w262:bool)
              }
              n150 = case shown="False" w231 {
                tunnel: w230 -> [_ w245]
                tunnel: w229 -> [_ w247]
                frame False {
                }
                frame True {
                  n151 = Bundle By Name(cluster=w247, "Actions"=Quick_Stack_Actions."Abort") -> (w244:T1)
                  n152 = Send Notification(notification=w244, notifier=w245) -> ()  [unwired: 1 in, 2 out]
                }
              }
              n153 = Select(t=Quick_Stack_Marked_Areas_Actions."Reset Path", s=w231, f=Quick_Stack_Marked_Areas_Actions."Switch") -> (s? t:f=w240:T3)
            }
            frame "Switch" {
              n154 = property on="Marked Positions" class="MCListbox (strict)"() -> ("Value"=w280:i32)  [unwired: 2 in, 2 out]
              n155 = Array Size(array=w276) -> (size(s)=w279:i32)
              n156 = Increment(x=w280) -> (x+1=w275:i32)
              n157 = Greater Or Equal?(x=w275, y=w279) -> (x >= y?=w269:bool)
              n158 = case shown="True" w269 {
                tunnel: w275 -> [w283 _]
                tunnel: [w283 0] -> w274
                tunnel: w273 -> [w282 w285]
                tunnel: [w282 w284] -> w271
                frame False {
                }
                frame True {
                  n159 = Increment(x=w285) -> (x+1=w284:u16)
                }
              }
              n160 = Equal?(x="Number of Cycles", y=w271) -> (x = y?=w270:bool)
              n161 = property on="Marked Positions" class="MCListbox (strict)"("Value"=w274) -> ()  [unwired: 2 in, 2 out]
              n162 = Implies(1:w270, 2:w269) -> (0:w266:bool)
              n163 = Select(t=Quick_Stack_Marked_Areas_Actions."Move to Position" ("y"), s=w266, f=Quick_Stack_Marked_Areas_Actions."Delay" ("y")) -> (s? t:f=w265:T3)
              n164 = Select(t=Quick_Stack_Marked_Areas_Actions."Reset Path" ("y"), s=w270, f=w265) -> (s? t:f=w277:T3)
            }
            frame "Delay" {
              n165 = Multiply(x="Cycle Delay (s)", y=u32 10) -> (x*y=w297:u32)
              n166 = To Long Integer(number=w297) -> (32bit integer=w298:i32)
              n167 = for {
                N: w298 -> [_]
                tunnel: w292 -> [w310]
                tunnel: [w308] -> w291
                tunnel: w290 -> [w303]
                tunnel: [w303] -> w289
                i -> [w307]
                stop <- w308 stop-if-true
                n168 = To Double Precision Float(number=w307) -> (double precision float=w306:dbl)
                n169 = Get Notifier Status(notifier=w310) -> (current notification=w309:T3)  [unwired: 1 in, 4 out]
                n170 = Equal?(x=w309, y=Quick_Stack_Marked_Areas_Actions."Abort") -> (x = y?=w308:bool)
                n171 = Divide(x=w306, y=10.0) -> (x/y=→"Current Delay Time (s)":dbl)
                n172 = Wait (ms)(milliseconds to wait=u32 100) -> ()  [unwired: 1 out]
              }
              n173 = Increment(x=w289) -> (x+1=→"Current Cycle":u16)
              n174 = Select(t=Quick_Stack_Marked_Areas_Actions."Reset Path" ("y"), s=w291, f=Quick_Stack_Marked_Areas_Actions."Move to Position" ("y")) -> (s? t:f=w293:T3)
            }
            frame "Reset Path" {
              n175 = Get Notifier Status(notifier=w318) -> (notifier out=w317:refnum<notifier>, current notification=w316:T1)  [unwired: 1 in, 3 out]
              n176 = Bundle By Name(cluster=w316, "Actions"=Quick_Stack_Actions."Idle", "Save Path"=w313) -> (w314:T1)
              n177 = Send Notification(notification=w314, notifier=w317) -> ()  [unwired: 1 in, 2 out]
            }
            frame "Remove Position" {
              n178 = property on="Marked Positions" class="MCListbox (strict)"() -> ("Value"=w327:i32)  [unwired: 2 in, 2 out]
              n179 = Delete From Array(array=w325, length=1, index=w327) -> (array with subset deleted=w324:T1[])  [unwired: 1 out]
            }
            frame "Clear All" {
            }
            frame "Quit" {
              n180 = Release Notifier(notifier=w339) -> ()  [unwired: 2 in, 3 out]
              n181 = Release Notifier(notifier=w338) -> ()  [unwired: 2 in, 3 out]
            }
          }
        }
      }
      n182 = local write "Quit"(w60) -> ()
    }
    frame Error {
    }
  }
  n183 = property class="VI"(reference=w14) -> (reference out=w23:refnum<vi>, "Panel"=w15:refnum<vi>)  [unwired: 1 in, 1 out]
  n184 = property class="Pnl"(reference=w15) -> ("Decos[]"=w13:refnum<vi>[], "Panes[]"=w19:refnum<vi>[])  [unwired: 1 in, 2 out]
  n185 = Array Size(array=w13) -> (size(s)=w11:i32)
  n186 = Decrement(x=w11) -> (x-1=w12:i32)
  n187 = Index Array(array=w19, index=0) -> (element=w18:refnum<vi>)
  n188 = Index Array(array=w13, index=w12) -> (element=w21:refnum<vi>)
  n189 = property class="VI"(reference=w23) -> (reference out=w25:refnum<vi>, "Front Panel.PanelBounds"=w26:T12)  [unwired: 1 in, 1 out]
  n190 = property class="Decor"(reference=w21) -> ("Bounds"=w24:T13)  [unwired: 1 in, 2 out]
  n191 = property class="Pane"(reference=w18, "Origin"=T5 {"Horizontal"=0, "Vertical"=0}, "HorizScrollbarVisibility"=w22, "VertScrollbarVisibility"=w22) -> ()  [unwired: 1 in, 2 out]
  n192 = Unbundle By Name(w24) -> ("Width"=w29:u32, "Height"=w32:u32)
  n193 = control-ref of="Quit"() -> (w16:refnum<vi>)
  n194 = To Word Integer(number=w29) -> (16bit integer=w31:i16)
  n195 = To Word Integer(number=w32) -> ()  [unwired: 1 out]
  n196 = property class="Bool (strict)"(reference=w16) -> ("Height"=w34:u32, "Top"=w35:i32)  [unwired: 1 in, 2 out]
  n197 = Unbundle By Name(w26) -> ("Left"=w28:i16, "Top"=w39:i16)
  n198 = To Word Integer(number=w34) -> (16bit integer=w37:i16)
  n199 = To Word Integer(number=w35) -> (16bit integer=w38:i16)
  n200 = Add(x=w28, y=w31) -> (x+y=w30:i16)
  n201 = Compound Arithmetic op=ADD(w39, w37, w38, i16 12 ("y")) -> (w33:i16)
  n202 = Bundle By Name(cluster=w26, "Right"=w30, "Bottom"=w33) -> (w27:T12)
  n203 = property class="VI"(reference=w25, "Front Panel.PanelBounds"=w27) -> ()  [unwired: 1 in, 2 out]
